vi "Post-Build Action.vi"(5 "Files Generated by Build":path[](array[path]), 6 "Top Level/Always Included VIs":path[](array[path]), 7 "Destination Path":path, 8 "error in":errorcluster, 9 "Target Name":string, 10 "Build Specification Name":string, 11 "Project Path":path) -> (0 "error out":errorcluster)   [LabVIEW 2027]
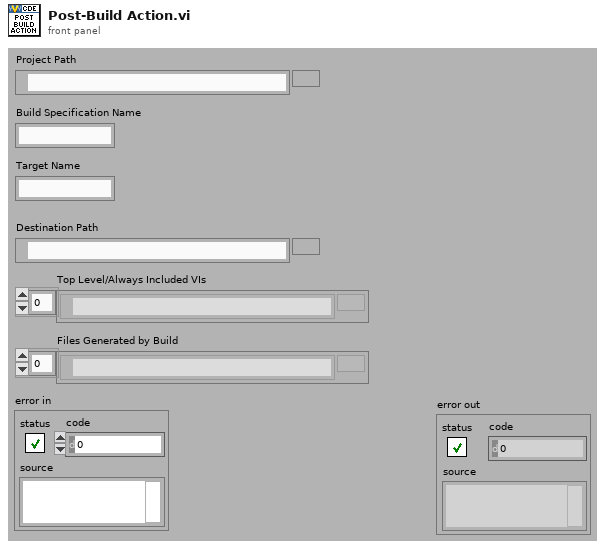
[diagram p1: front panel]
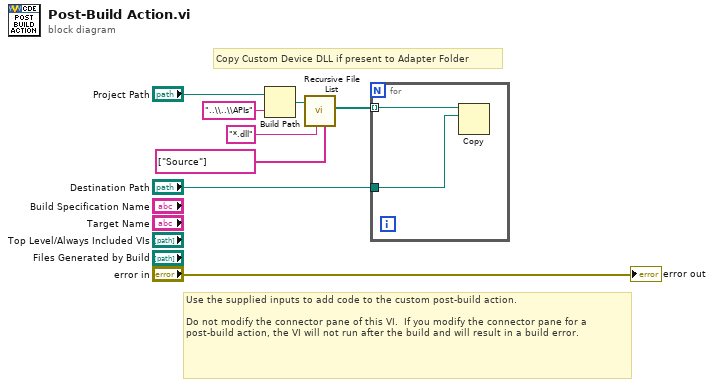
[diagram p0: block diagram]
diagram:
  # "Copy Custom Device DLL if present to Adapter Folder"
  # "Use the supplied inputs to add code to the custom post-build action.\n\nDo not modify the connector pane of this VI.  If you modify the connector pane for a post-build action, the VI will not run after the build and will result in a build error."
  n1 = Build Path(base path="Project Path", name or relative path="..\\..\\APIs") -> (appended path=w3:path)
  n2 = call <vilib>:"Recursive File List.vi"("Folders to Exclude"=string[] ["Source"], "pattern"="*.dll", "Folder Path"=w3) -> ("All Files in Dir"=w2:path[])  [unwired: 4 in, 4 out]
  n3 = for {
    tunnel: "Destination Path" -> [w10]
    tunnel: w2 -> [w9] mode=indexing
    n4 = Copy(10:w10, 11:w9) -> ()  [unwired: 3 in, 3 out]
  }
  "error out" <- "error in"
